vi "Check valid stack ID.vi"(6 "Is real run?":bool, 8 "error in (no error)":errorcluster, 11 "Stack in":refnum<class "Stack.lvclass">) -> (0 "error out":errorcluster, 1 "Non-empty part IDs?":bool, 2 "Valid module ID?":bool, 3 "Stack out":refnum<class "Stack.lvclass">, 5 "Non-empty assembly tray ID?":bool)   [LabVIEW 2021, in "Stack.lvclass"]
uses:
  Stack.lvclass
  Stack.lvclass/Stack.ctl
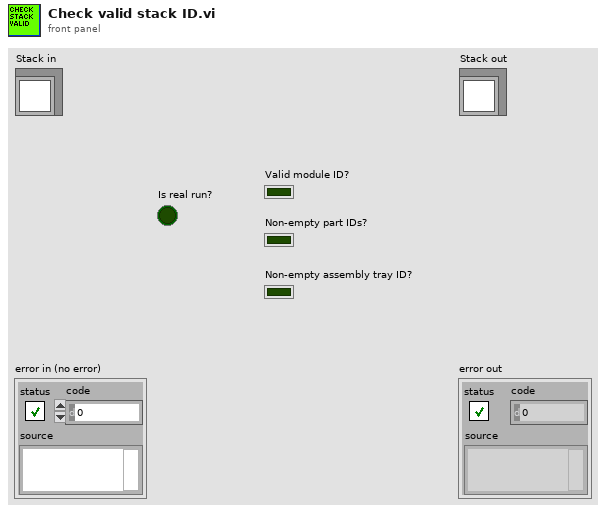
[diagram p1: front panel]
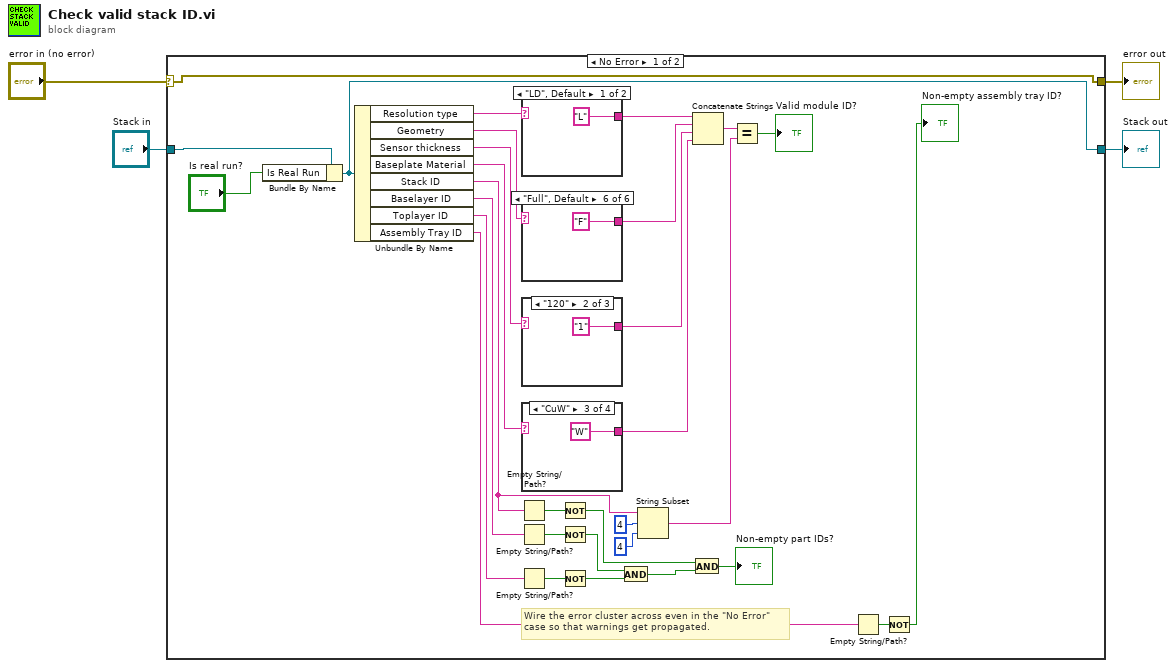
[diagram p0: block diagram]
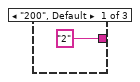
[diagram p2: hidden frame]
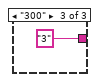
[diagram p3: hidden frame]
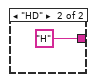
[diagram p4: hidden frame]
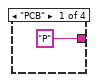
[diagram p5: hidden frame]
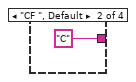
[diagram p6: hidden frame]
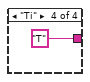
[diagram p7: hidden frame]
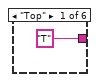
[diagram p8: hidden frame]
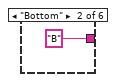
[diagram p9: hidden frame]
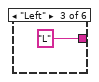
[diagram p10: hidden frame]
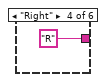
[diagram p11: hidden frame]
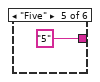
[diagram p12: hidden frame]
diagram:
  n1 = case shown="No Error" "error in (no error)" {
    selector: "error in (no error)" -> [w35 w52]
    tunnel: [w35 w52] -> w3
    tunnel: [w5 w51] -> w1
    tunnel: "Stack in" -> [w7 w51]
    frame No Error {
      # "Wire the error cluster across even in the \"No Error\"\ncase so that warnings get propagated."
      n2 = Bundle By Name(cluster=w7, "Is Real Run"="Is real run?") -> (w5:refnum<class "Stack.lvclass">)
      n3 = Unbundle By Name(w5) -> ("Resolution type"=w34:string, "Geometry"=w33:string, "Sensor thickness"=w32:string, "Baseplate Material"=w31:string, "Stack ID"=w12:string, "Baselayer ID"=w21:string, "Toplayer ID"=w20:string, "Assembly Tray ID"=w13:string)
      n4 = Empty String/Path?(string/path=w12) -> (empty?=w11:bool)
      n5 = Empty String/Path?(string/path=w21) -> (empty?=w19:bool)
      n6 = Empty String/Path?(string/path=w20) -> (empty?=w18:bool)
      n7 = case shown="\"LD\", Default" w34 {
        tunnel: ["L" "H"] -> w30
        frame "LD", Default {
        }
        frame "HD" {
        }
      }
      n8 = case shown="\"Full\", Default" w33 {
        tunnel: ["T" "B" "L" "R" "5" "F"] -> w29
        frame "Top" {
        }
        frame "Bottom" {
        }
        frame "Left" {
        }
        frame "Right" {
        }
        frame "Five" {
        }
        frame "Full", Default {
        }
      }
      n9 = case shown="\"120\"" w32 {
        tunnel: ["2" "1" "3"] -> w28
        frame "200", Default {
        }
        frame "120" {
        }
        frame "300" {
        }
      }
      n10 = case shown="\"CuW\"" w31 {
        tunnel: ["P" "C" "W" "T"] -> w27
        frame "PCB" {
        }
        frame "CF ", Default {
        }
        frame "CuW" {
        }
        frame "Ti" {
        }
      }
      n11 = Not(x=w11) -> (.not. x?=w10:bool)
      n12 = Not(x=w19) -> (.not. x?=w16:bool)
      n13 = Not(x=w18) -> (.not. x?=w17:bool)
      n14 = And(x=w16, y=w17) -> (x .and. y?=w9:bool)
      n15 = String Subset(string=w12, offset (0)=4, length (rest)=4 ("length (rest)")) -> (substring=w22:string)
      n16 = And(x=w10, y=w9) -> (x .and. y?=→"Non-empty part IDs?":bool)
      n17 = Concatenate Strings(w30, w29, w28, w27) -> (w26:string)
      n18 = Equal?(x=w26, y=w22) -> (x = y?=→"Valid module ID?":bool)
      n19 = Empty String/Path?(string/path=w13) -> (empty?=w15:bool)
      n20 = Not(x=w15) -> (.not. x?=→"Non-empty assembly tray ID?":bool)
    }
    frame Error {
    }
  }
  "error out" <- w3
  "Stack out" <- w1
